vi "GPIB_Address.vi"() -> ()   [LabVIEW 2024]
panel:
  out "String":string
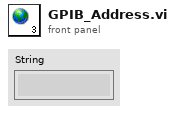
[diagram p1: front panel]
diagram:
